vi "Serial Receive.vi"(6 "ready for output":bool, 7 "data sampling edge":enum16{"rising", "falling"}(ring)=enum."falling", 8 "transfer length":u8, 9 "force stop (F)":bool, 10 "start transfer":bool, 11 "signals in":cluster{"clock":bool, "data":bool}) -> (0 "transfer done":bool, 1 "output valid":bool, 3 "sample out":u32)   [LabVIEW 2013, in "I2S-TDM.lvlib"]
uses:
  I2S-TDM.lvlib
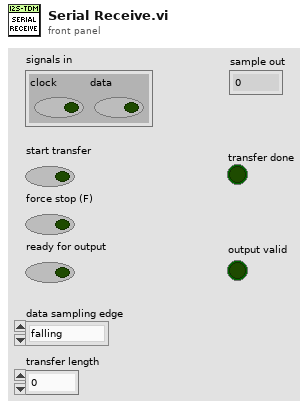
[diagram p1: front panel]
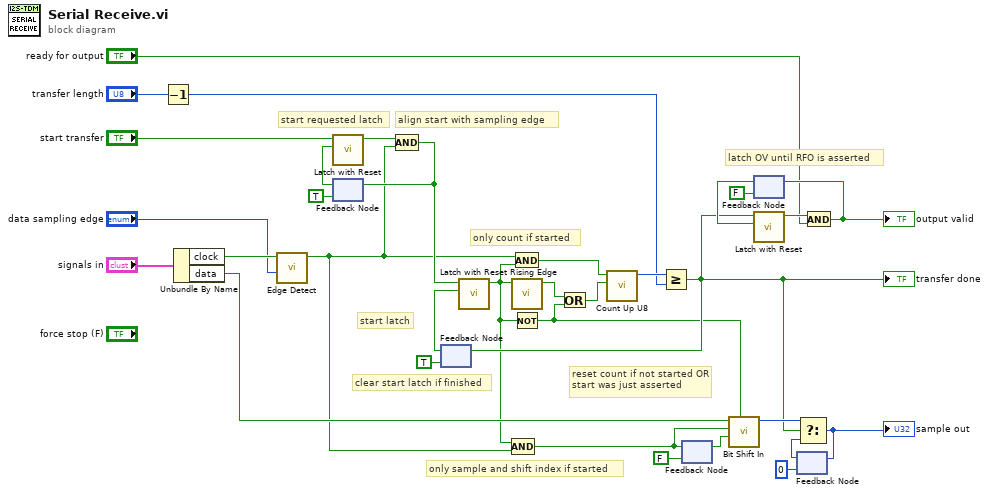
[diagram p0: block diagram]
diagram:
  # "clear start latch if finished"
  # "start latch"
  # "only sample and shift index if started"
  # "reset count if not started OR start was just asserted"
  # "only count if started"
  # "latch OV until RFO is asserted"
  # "align start with sampling edge"
  # "start requested latch"
  n1 = Decrement(x="transfer length") -> (x-1=w21:u8)
  n2 = Unbundle By Name("signals in") -> ("clock"=w33:bool, "data"=w25:bool)
  n3 = call "Edge Detect.vi"("edge (rising)"="data sampling edge", "signal in"=w33) -> ("edge detected?"=w2:bool)  [unwired: 9 in]
  n4 = feedback #1(TRUE) -> (w31:bool)
  n5 = call "Latch with Reset.vi"("reset"=w31, "signal"="start transfer") -> ("latched signal"=w24:bool)  [unwired: 9 in]
  n6 = Compound Arithmetic op=AND(w24, w2) -> (w23:bool)
  n7 = feedback-in #1(w23) -> ()
  n8 = feedback #2(TRUE) -> (w19:bool)
  n9 = call "Latch with Reset.vi"("reset"=w19, "signal"=w23) -> ("latched signal"=w3:bool)  [unwired: 9 in]
  n10 = And(x=w2, y=w3) -> (x .and. y?=w14:bool)
  n11 = call "Rising Edge.vi"("signal in"=w3) -> ("rising edge?"=w13:bool)  [unwired: 10 in]
  n12 = Not(x=w3) -> (.not. x?=w11:bool)
  n13 = Compound Arithmetic op=AND(w3, w2) -> (w1:bool)
  n14 = Or(x=w13, y=w11) -> (x .or. y?=w12:bool)
  n15 = call "Count Up U8.vi"("reset (F)"=w12, "increment"=w14) -> ("count"=w22:u8)  [unwired: 9 in]
  n16 = Greater Or Equal?(x=w22, y=w21) -> (x >= y?=w15:bool)
  "transfer done" <- w15
  n17 = feedback-in #2(w15) -> ()
  n18 = feedback #3(FALSE ("edge detected?")) -> (w29:bool)
  n19 = feedback-in #3(w1) -> ()
  n20 = call "Bit Shift In.vi"("reset"=w11, "shift index"=w29, "sample bit"=w1, "data bit in"=w25) -> ("sample"=w26:u32)  [unwired: 7 in]
  n21 = feedback #4(FALSE) -> (w16:bool)
  n22 = call "Latch with Reset.vi"("reset"=w16, "signal"=w15) -> ("latched signal"=w17:bool)  [unwired: 9 in]
  n23 = feedback #5(u32 0 ("sample")) -> (w27:u32)
  n24 = Select(t=w26, s=w15, f=w27) -> (s? t:f=w10:u32)
  "sample out" <- w10
  n25 = feedback-in #5(w10) -> ()
  n26 = And(x=w17, y="ready for output") -> (x .and. y?=w9:bool)
  "output valid" <- w9
  n27 = feedback-in #4(w9) -> ()
